vi "Result Display.vi"(8 "error in (no error)":errorcluster, 9 "Display ON/OFF":bool, 11 "Result":T1) -> (0 "error out":errorcluster, 3 "Result Display":picture)   [LabVIEW 2018, in "Pass Fail Display.lvlib"]
doc: "This VI displays the image with the text 'Serial Number PASS' or 'Serial Number OFF' on the SN stat DSP indicator, according to the SN Status and Display ON/OFF controls."
uses:
  Pass Fail Display.lvlib
  Result--enum.ctl
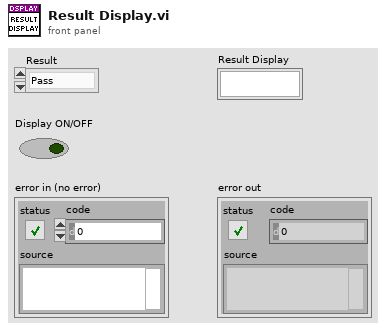
[diagram p1: front panel]
types:
  T1 = typedef "Pass Fail Display.lvlib/Result--enum.ctl" = enum16{"Pass", "Fail"}
  T2 = typedef "imagedata.ctl" = cluster{"image type":i32, "image depth":i32, "image":u8[], "mask":u8[], "colors":u32[], "Rectangle":cluster{"left":i16, "top":i16, "right":i16, "bottom":i16}}
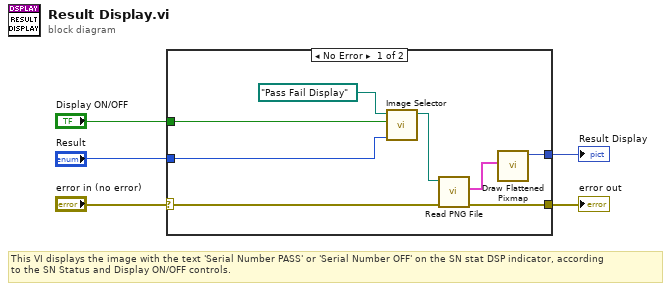
[diagram p0: block diagram]
diagram:
  # "This VI displays the image with the text 'Serial Number PASS' or 'Serial Number OFF' on the SN stat DSP indicator, according\nto the SN Status and Display ON/OFF controls."
  n1 = case shown="No Error" "error in (no error)" {
    selector: "error in (no error)" -> [w6 w14]
    tunnel: "Result" -> [w7 _]
    tunnel: [w13 _] -> w1
    tunnel: [w12 w14] -> w5
    tunnel: "Display ON/OFF" -> [w9 _]
    frame No Error {
      n2 = call "Image Selector.vi"("Result"=w7, "Display ON/OFF"=w9, "Relative folder path name"=path "Pass Fail Display") -> ("Path to PNG file"=w10:path)  [unwired: 8 in]
      n3 = call <vilib>:"Read PNG File.vi"("error in (no error)"=w6, "path to PNG file"=w10) -> ("error out"=w12:errorcluster, "image data"=w11:T2)  [unwired: 7 in, 1 out]
      n4 = call <vilib>:"Draw Flattened Pixmap.vi"("image data"=w11) -> ("new picture"=w13:picture)  [unwired: 8 in]
    }
    frame Error {
    }
  }
  "error out" <- w5
  "Result Display" <- w1
